vi "Lire donnees generales prog MODBUS EPC.vi"(3 "error in (no error)":errorcluster caption="entrée d'erreur (pas d'erreur)", 4 "N° prog":u8 caption="N° programme", 5 "Adresse régulateur":u8, 6 "Port COM":refnum<visa-resource-name>) -> (0 "error out":errorcluster caption="entrée d'erreur (pas d'erreur)", 1 "données générales":u16[](array[numeric]), 2 "Programmation données":cluster{"chaîne o":string, dbl}[](array[cluster]))   [LabVIEW 2022 SP3]
uses:
  Variables globales/Variables glob EUROTHERM.vi
panel:
  out "Data 2 (U16)":u16[][](array[numeric])
  # "lecture données générales"
  # "unités rampe"
  # "unités palier"
  # "nb cycles"
  # "type fin"
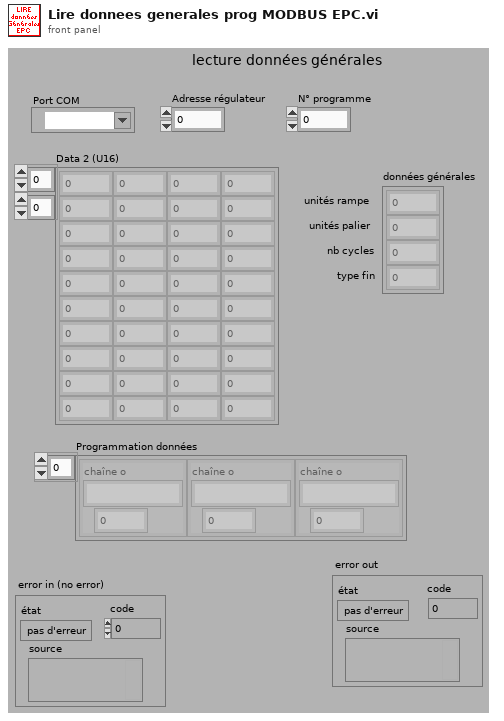
[diagram p1: front panel]
types:
  T1 = typedef "Semaphore RefNum" = refnum<k1>
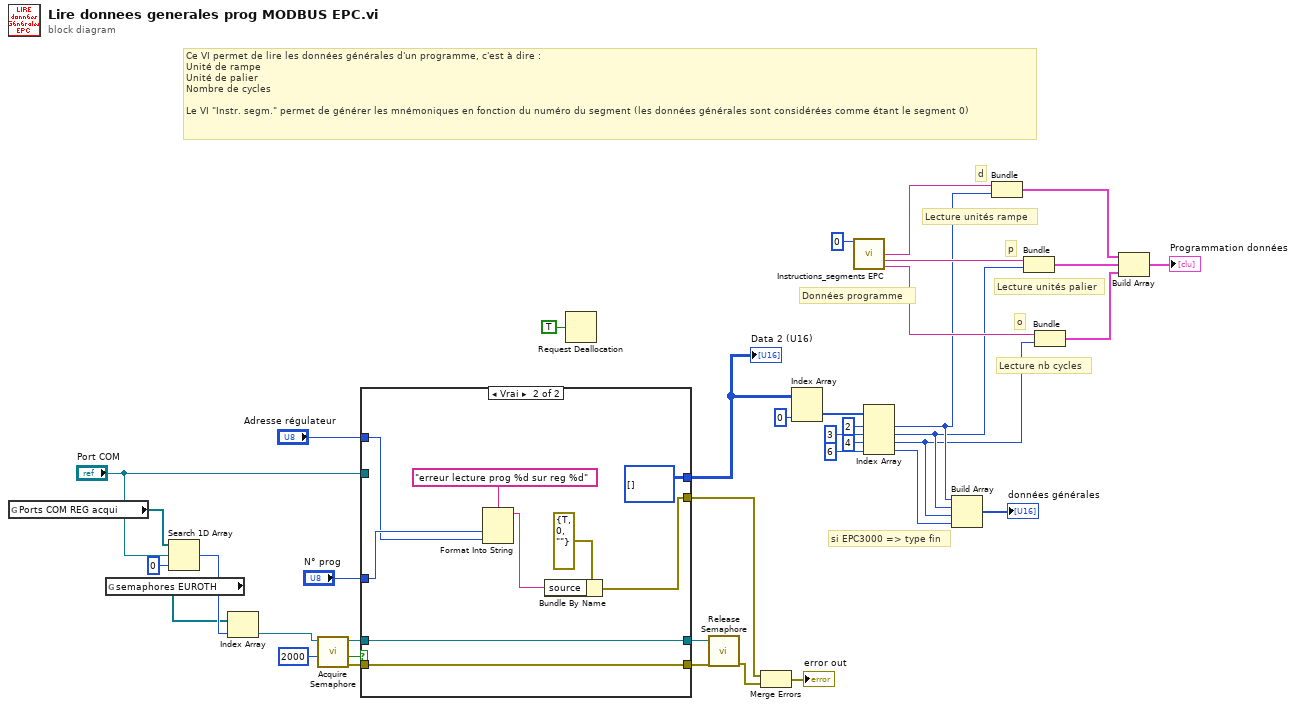
[diagram p0: block diagram]
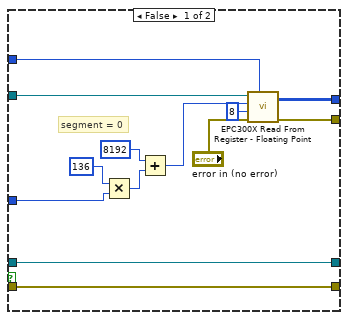
[diagram p2: hidden frame]
diagram:
  # "si EPC3000 => type fin"
  # "Lecture nb cycles"
  # "o"
  # "Lecture unités palier"
  # "p"
  # "Lecture unités rampe"
  # "d"
  # "Ce VI permet de lire les données générales d'un programme, c'est à dire :\nUnité de rampe\nUnité de palier\nNombre de cycles\n\nLe VI \"Instr. segm.\" permet de générer les mnémoniques en fonction du numéro du segment (les données générales sont considérées comme étant le segment 0)"
  # "Données programme"
  n1 = global read "Variables glob EUROTHERM.vi" "Ports COM REG acqui"() -> (w14:refnum<visa-resource-name>[])
  n2 = global read "Variables glob EUROTHERM.vi" "semaphores EUROTH"() -> (w15:T1[])
  n3 = Search 1D Array(1D array=w14, element="Port COM", start index (0)=0 ("indice de départ (0)")) -> (index of element=w16:i32)
  n4 = Index Array(array=w15, index=w16) -> (element=w11:T1)
  n5 = call <vilib>:"Acquire Semaphore.vi"("ms timeout (-1)"=2000, "semaphore"=w11) -> ("error out"=w7:errorcluster, "timed out"=w9:bool, "semaphore out"=w8:T1)  [unwired: 3 in]
  n6 = case shown="Vrai" w9 {
    tunnel: "N° prog" -> [w48 w53]
    tunnel: [w47 u16[][] [] ("Data 2 (U16)")] -> w22
    tunnel: [w44 w55] -> w3
    tunnel: "Port COM" -> [w42 _]
    tunnel: w8 -> [w41 w57]
    tunnel: w7 -> [w40 w56]
    tunnel: [w41 w57] -> w5
    tunnel: [w40 w56] -> w4
    tunnel: "Adresse régulateur" -> [w39 w52]
    frame False {
      # "segment = 0"
      n7 = Multiply(x=u64 136, y=w48) -> (x*y=w50:u64)
      n8 = Add(x=u64 8192, y=w50) -> (x+y=w46:u64)
      n9 = call "EPC300X Read From Register - Floating Point.vi"("Unit Address (1)"=w39, "error in (no error)"="error in (no error)", "Num Of Reg (1)"=u16 8, "Register Address (0)"=w46, "VISA session"=w42) -> ("error out"=w44:errorcluster, "Data 2 (U16)"=w47:u16[][])  [unwired: 1 in, 4 out]
    }
    frame True {
      n10 = Format Into String(format string="erreur lecture prog %d sur reg %d" ("chaîne de format"), w53, w52) -> (resulting string=w60:string)  [unwired: 2 in, 1 out]
      n11 = Bundle By Name(cluster=errorcluster {"status"=TRUE, "code"=0, "source"=""} ("error out"), "source"=w60) -> (w55:errorcluster)
    }
  }
  "Data 2 (U16)" <- w22
  n12 = Request Deallocation(TRUE ("flag")) -> ()
  n13 = call <vilib>:"Release Semaphore.vi"("error in (no error)"=w4, "semaphore"=w5) -> ("error out"=w6:errorcluster)  [unwired: 4 in, 1 out]
  n14 = Merge Errors(w3, w6) -> (→"error out":errorcluster)
  n15 = Index Array(array=w22, index (col)=0 ("indice (ligne)")) -> (element=w24:u16[])  [unwired: 1 in]
  n16 = call "Instructions_segments EPC.vi"("Numéro de segment"=i8 0) -> ("chaîne d"=w33:string, "chaîne p"=w32:string, "chaîne o"=w31:string)  [unwired: 10 in, 2 out]
  n17 = Index Array(array=w24, index #1=2 ("indice"), index #2=3 ("indice"), index #3=4 ("indice"), index #4=6 ("indice")) -> (element #1=w20:u16, element #2=w19:u16, element #3=w18:u16, element #4=w17:u16)
  n18 = Build Array(w20, w19, w18, w17) -> (→"données générales":u16[])
  n19 = Bundle("chaîne d"=w33, w20) -> (w35:cluster{"chaîne d":string, u16})  [unwired: 1 in]
  n20 = Bundle("chaîne p"=w32, w19) -> (w36:cluster{"chaîne p":string, u16})  [unwired: 1 in]
  n21 = Bundle("chaîne o"=w31, w18) -> (w37:cluster{"chaîne o":string, u16})  [unwired: 1 in]
  n22 = Build Array(w35, w36, w37) -> (→"Programmation données":cluster{"chaîne o":string, u16}[])
